vi "SPARK Get Analog Sensor Config.vi"   [LabVIEW 2023]
doc: "Get the configuration of the analog sensor connected to the data port of the SPARK."
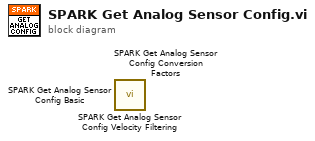
[diagram p0: block diagram]
diagram:
  n1 = call <vilib>:"SPARK Get Analog Sensor Config Velocity Filtering.vi"() -> ()  [unwired: 8 in, 4 out]
  n2 = call <vilib>:"SPARK Get Analog Sensor Config Conversion Factors.vi"() -> ()  [unwired: 8 in, 4 out]
  n3 = call <vilib>:"SPARK Get Analog Sensor Config Basic.vi"() -> ()  [unwired: 8 in, 4 out]
